vi "Assert Equal Value_Variant.vi"(4 "Execution time (s)":dbl=-1.0, 5 "Assert Only? (F)":bool, 6 "error code (1)":i32=1, 7 "Label":string, 8 "error in (no error)":errorcluster, 9 "Register with caller test (F)":bool, 10 "Actual":variant, 11 "Expected":variant) -> (0 "error out":errorcluster, 2 "Properties.Assert":refnum<class "Properties.Assert.lvclass">)   [LabVIEW 2013, in "Caraya.lvlib" / "Assert.lvclass"]
doc: "Generates an error if the input condition is not met.\n\nThis method compares the value of the inputs, irrespective of the type representation.\nAsserts TRUE if input values are equal.\nAsserts FALSE otherwise.\n\nex: Two integer inputs of equal value but of different type representation (U8 and I32) will assert TRUE."
uses:
  Assert.lvclass
  Properties.Assert/Properties.Assert.lvclass
  Properties/Properties.lvclass
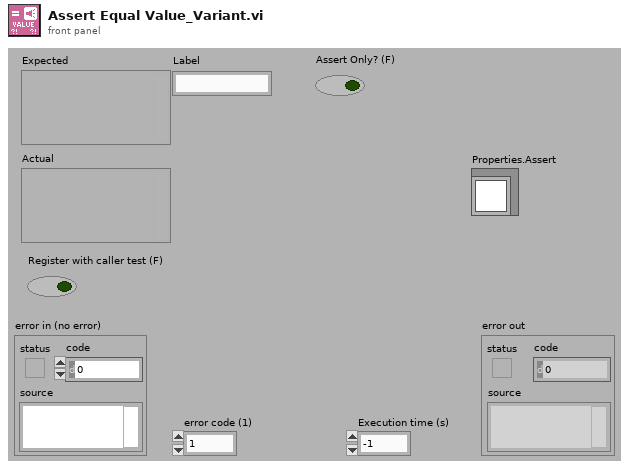
[diagram p1: front panel]
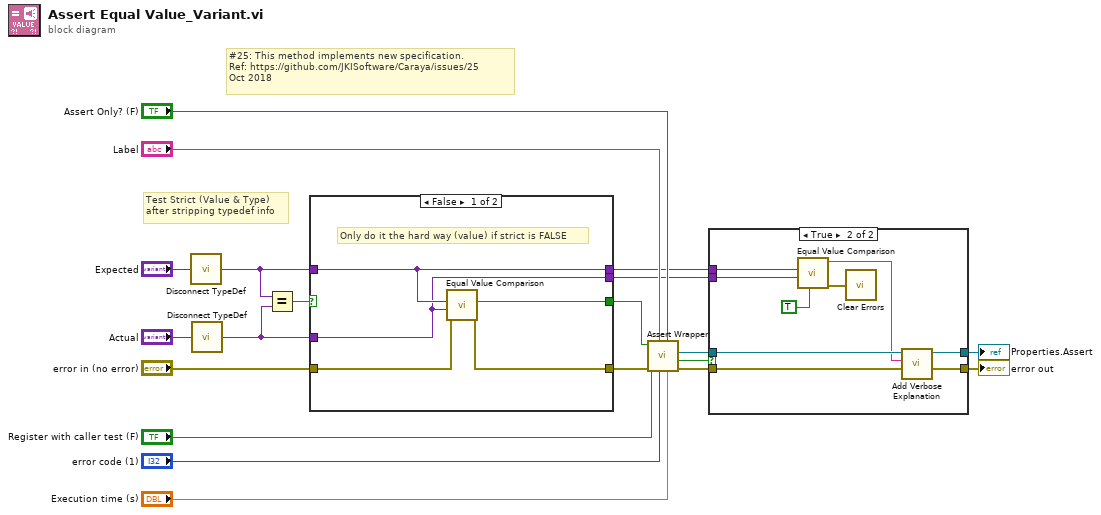
[diagram p0: block diagram]
diagram:
  # "Test Strict (Value & Type)\nafter stripping typedef info"
  # "#25: This method implements new specification.\nRef: https://github.com/JKISoftware/Caraya/issues/25\nOct 2018"
  n1 = call "Disconnect TypeDef.vi"("Variant"="Expected") -> ("Variant Out"=w14:variant)
  n2 = call "Disconnect TypeDef.vi"("Variant"="Actual") -> ("Variant Out"=w12:variant)
  n3 = Equal?(x=w14, y=w12) -> (x = y?=w16:bool)
  n4 = case shown="False" w16 {
    selector: w16 -> [_ w29]
    tunnel: [w25 w29] -> w17
    tunnel: "error in (no error)" -> [w24 w28]
    tunnel: [w23 w28] -> w10
    tunnel: w14 -> [w22 w27]
    tunnel: w12 -> [w21 w26]
    tunnel: [w22 w27] -> w6
    tunnel: [w21 w26] -> w5
    frame False {
      # "Only do it the hard way (value) if strict is FALSE"
      n5 = call "Equal Value Comparison.vi"("error in (no error)"=w24, "Actual"=w21, "Expected"=w22) -> ("error out"=w23:errorcluster, "Equal Values?"=w25:bool)  [unwired: 6 in, 1 out]
    }
    frame True {
    }
  }
  n6 = call "Assert Wrapper.vi"("Execution time (s)"="Execution time (s)", "Assert Only? (F)"="Assert Only? (F)", "error code (1)"="error code (1)", "Label"="Label", "error in (no error)"=w10, "Register with caller test (F)"="Register with caller test (F)", "Assert?"=w17) -> ("error out"=w9:errorcluster, "Verbose"=w4:bool, "Properties.Assert"=w2:refnum<class "Properties.Assert.lvclass">)  [unwired: 1 in, 1 out]
  n7 = case shown="True" w4 {
    tunnel: [w31 w33] -> w7
    tunnel: w9 -> [w31 w34]
    tunnel: w6 -> [_ w40]
    tunnel: w5 -> [_ w39]
    tunnel: w2 -> [w30 w36]
    tunnel: [w30 w32] -> w1
    frame False {
    }
    frame True {
      n8 = call "Equal Value Comparison.vi"("verbose? (F)"=TRUE, "Actual"=w39, "Expected"=w40) -> ("error out"=w37:errorcluster, "Verbose output"=w35:string)  [unwired: 6 in, 1 out]
      n9 = call <vilib>:"Clear Errors.vi"("error in (no error)"=w37) -> ()  [unwired: 6 in, 1 out]
      n10 = call "Add Verbose Explanation.vi"("error in (no error)"=w34, "Verbose Explanation"=w35, "Properties"=w36) -> ("error out"=w33:errorcluster, "Properties"=w32:refnum<class "Properties.Assert.lvclass">)  [unwired: 7 in]
    }
  }
  "error out" <- w7
  "Properties.Assert" <- w1
